vi "Error_Handling.vi"(4 "8":errorcluster={"status"=FALSE, "code"=5000, "source"=""} caption="3", 5 "1":errorcluster={"status"=FALSE, "code"=5000, "source"=""}, 6 "7":errorcluster={"status"=FALSE, "code"=5000, "source"=""} caption="3", 7 "2":errorcluster={"status"=FALSE, "code"=5000, "source"=""}, 8 "6":errorcluster={"status"=FALSE, "code"=5000, "source"=""} caption="3", 9 "5":errorcluster={"status"=FALSE, "code"=5000, "source"=""} caption="3", 10 "4":errorcluster={"status"=FALSE, "code"=5000, "source"=""} caption="3", 11 "3":errorcluster={"status"=FALSE, "code"=5000, "source"=""}) -> (0 "Error OUT":errorcluster caption="s? t:f")   [LabVIEW 2019]
panel:
  out "連結文字列":string
  out "final string":string
  out "長さ":i32
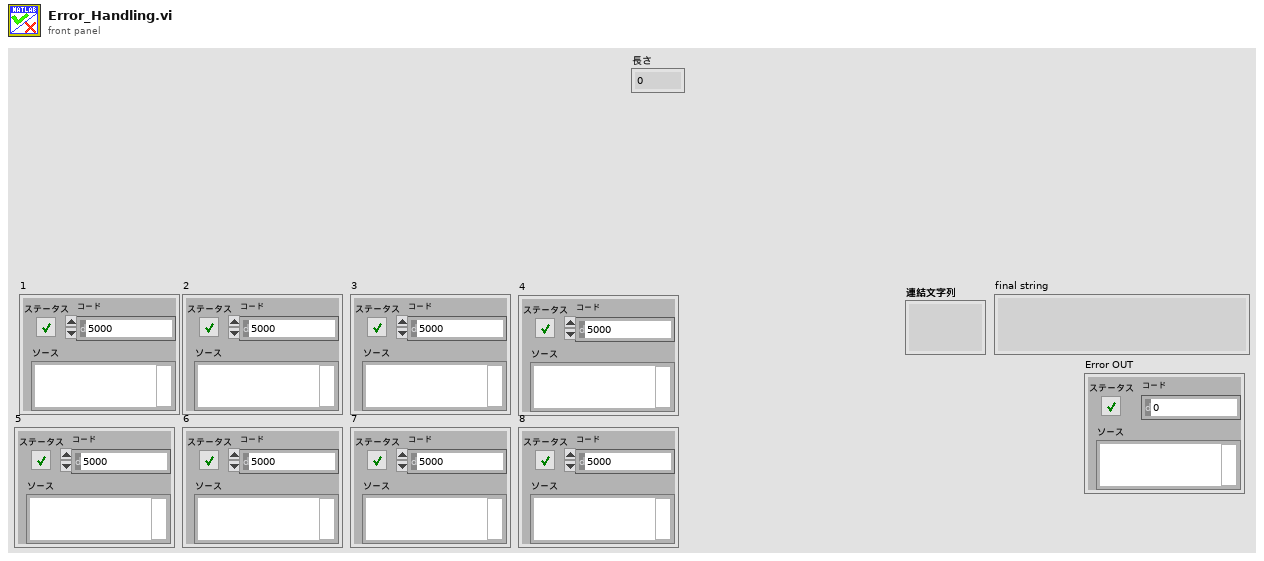
[diagram p1: front panel]
types:
  T1 = cluster{"1":errorcluster, "2":errorcluster, "3":errorcluster, "4":errorcluster, "5":errorcluster, "6":errorcluster, "7":errorcluster, "8":errorcluster}
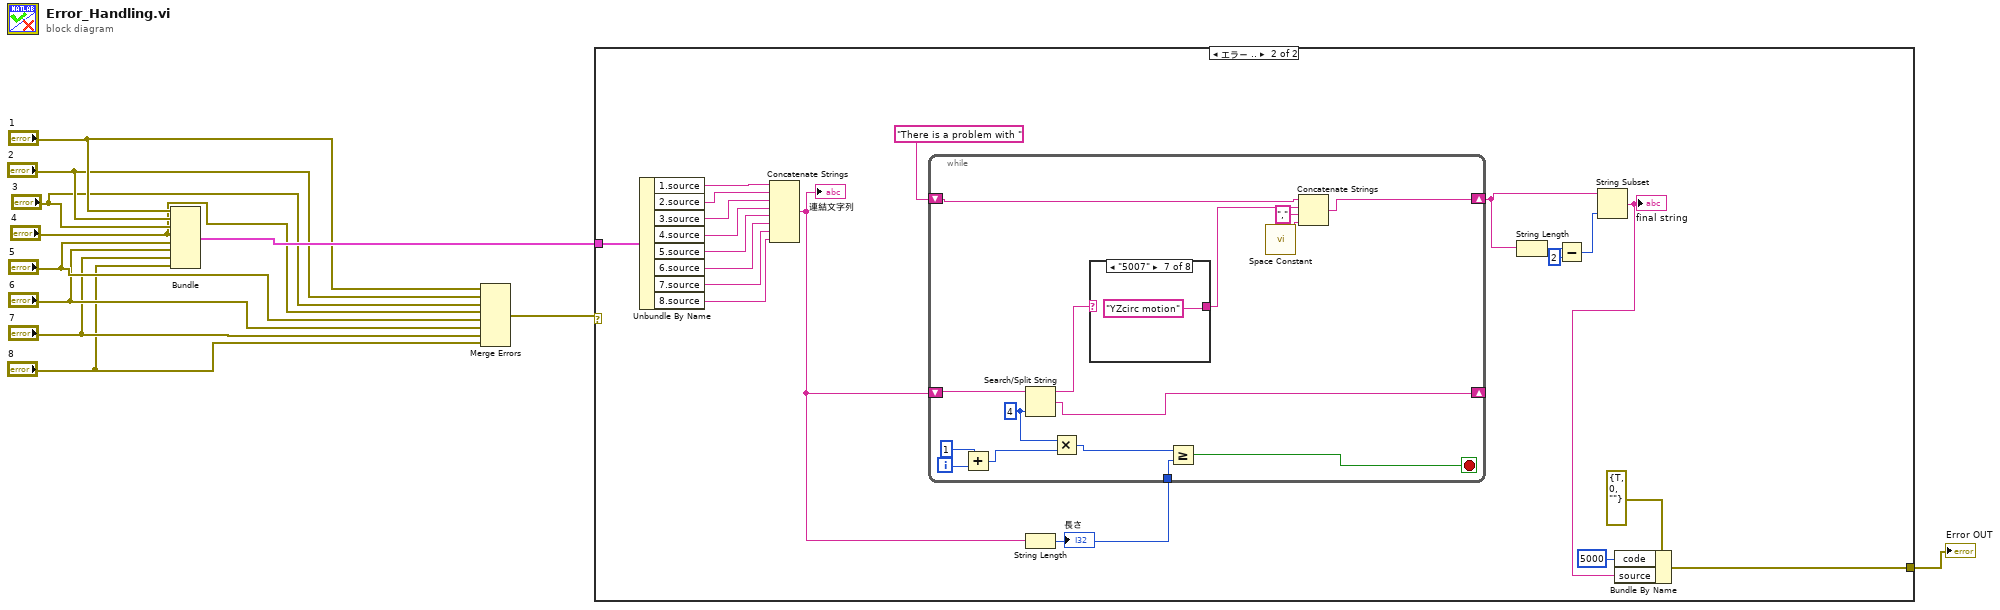
[diagram p0: block diagram]
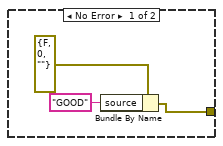
[diagram p2: hidden frame]
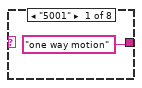
[diagram p3: hidden frame]
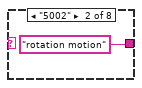
[diagram p4: hidden frame]
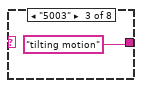
[diagram p5: hidden frame]
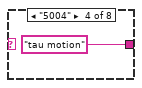
[diagram p6: hidden frame]
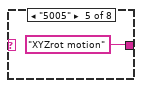
[diagram p7: hidden frame]
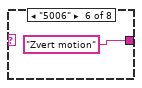
[diagram p8: hidden frame]
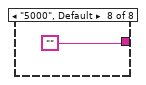
[diagram p9: hidden frame]
diagram:
  n1 = Bundle("1"="1", "2"="2", "3"="3", "4"="4", "5"="5", "6"="6", "7"="7", "8"="8") -> (w11:T1)  [unwired: 1 in]
  n2 = Merge Errors("1", "2", "3", "4", "5", "6", "7", "8") -> (w2:errorcluster)
  n3 = case shown="エラー .." w2 {
    tunnel: w11 -> [_ w24]
    tunnel: [w12 w15] -> w1
    frame No Error {
      n4 = Bundle By Name(cluster=errorcluster {"status"=FALSE, "code"=0, "source"=""} ("エラー定数"), "source"="GOOD") -> (w12:errorcluster)
    }
    frame Error {
      n5 = Unbundle By Name(w24) -> ("1.source"=w34:string, "2.source"=w33:string, "3.source"=w32:string, "4.source"=w20:string, "5.source"=w19:string, "6.source"=w18:string, "7.source"=w17:string, "8.source"=w16:string)
      n6 = Concatenate Strings(w34, w33, w32, w20, w19, w18, w17, w16) -> (w25:string)
      "連結文字列" <- w25
      n7 = String Length(string=w25) -> (length=w30:i32)
      "長さ" <- w30
      n8 = while {
        shift-right: [w48] -> _
        shift-left: w25 -> [w49]
        shift-right: [w35] -> w29
        shift-left: "There is a problem with " ("文字列") -> [w37]
        tunnel: w30 -> [w45]
        i -> [w47]
        stop <- w44 stop-if-true
        w43 = 4 ("オフセット (0)")
        n9 = Add(x=1, y=w47) -> (x+y=w42:i32)
        n10 = Search/Split String(string=w49, offset (0)=w43) -> (substring before match=w40:string, match + rest of string=w48:string)  [unwired: 1 in, 1 out]
        n11 = Multiply(x=w43, y=w42) -> (x*y=w41:i32)
        n12 = case shown="\"5007\"" w40 {
          tunnel: ["one way motion" "rotation motion" "tilting motion" "tau motion" "XYZrot motion" "Zvert motion" "YZcirc motion" ""] -> w36
          frame "5001" {
          }
          frame "5002" {
          }
          frame "5003" {
          }
          frame "5004" {
          }
          frame "5005" {
          }
          frame "5006" {
          }
          frame "5007" {
          }
          frame "5000", Default {
          }
        }
        n13 = Greater Or Equal?(x=w41, y=w45) -> (x >= y?=w44:bool)
        n14 = call <vilib>:"Space Constant.vi"() -> ("String"=w38:string)
        n15 = Concatenate Strings(w37, w36, "," ("文字列"), w38) -> (w35:string)
      }
      n16 = String Length(string=w29) -> (length=w28:i32)
      n17 = Subtract(x=w28, y=2) -> (x-y=w26:i32)
      n18 = String Subset(string=w29, length (rest)=w26) -> (substring=w21:string)  [unwired: 1 in]
      "final string" <- w21
      n19 = Bundle By Name(cluster=errorcluster {"status"=TRUE, "code"=0, "source"=""} ("エラー定数"), "code"=5000, "source"=w21) -> (w15:errorcluster)
    }
  }
  "Error OUT" <- w1
